vi "TCT .vi"(11 "VISA resource name":refnum<visa-resource-name>) -> ()   [LabVIEW 2016]
uses:
  <vilib>/NI/Modbus Library/API/Wrapper/Create Serial Master.vi
  <vilib>/NI/Modbus Library/API/Master/Modbus Master.lvclass
  <vilib>/NI/Modbus Library/API/Wrapper/API Main.lvlib
panel:
  out "Mean Temp.":dbl
  out "Voltage":dbl
  in  "y":bool
  out "Average hot plate temp.":dbl
  out "Average cold plate temp.":dbl
  out "Average Thermal conductivity":dbl
  out "LHP":dbl
  out "UHP":dbl
  out "LCP":dbl
  out "UCP":dbl
  out "x < y? 3":bool
  out "x < y? 2":bool
  in  "upper and lower cold plate":dbl
  out "upper conductivity":dbl
  out "Lower conductivity":dbl
  in  "Thickness":u16
  out "current":u16
  out "x < y?":bool
  in  "set hot plate temp":dbl
  out "current":u16[](array[numeric])
  out "lower cold plate":dbl
  out "lower hot plate":dbl
  out "upper hot plate":dbl
  out "upper cold plate":dbl
  out "element 13":u16
  out "element 12":u16
  out "element 11":u16
  out "element 10":u16
  out "element 9":u16
  out "element 8":u16
  out "element 7":u16
  out "element 6":u16
  out "element 5":u16
  out "element 4":u16
  out "element 3":u16
  out "element 2":u16
  out "voltage":u16
  out "register values 13":u16[](array[numeric])
  out "register values 12":u16[](array[numeric])
  out "register values 11":u16[](array[numeric])
  out "register values 10":u16[](array[numeric])
  out "register values 9":u16[](array[numeric])
  out "register values 8":u16[](array[numeric])
  out "register values 7":u16[](array[numeric])
  out "register values 6":u16[](array[numeric])
  out "register values 5":u16[](array[numeric])
  out "register values 4":u16[](array[numeric])
  out "register values 3":u16[](array[numeric])
  out "register values 2":u16[](array[numeric])
  out "register values":u16[](array[numeric])
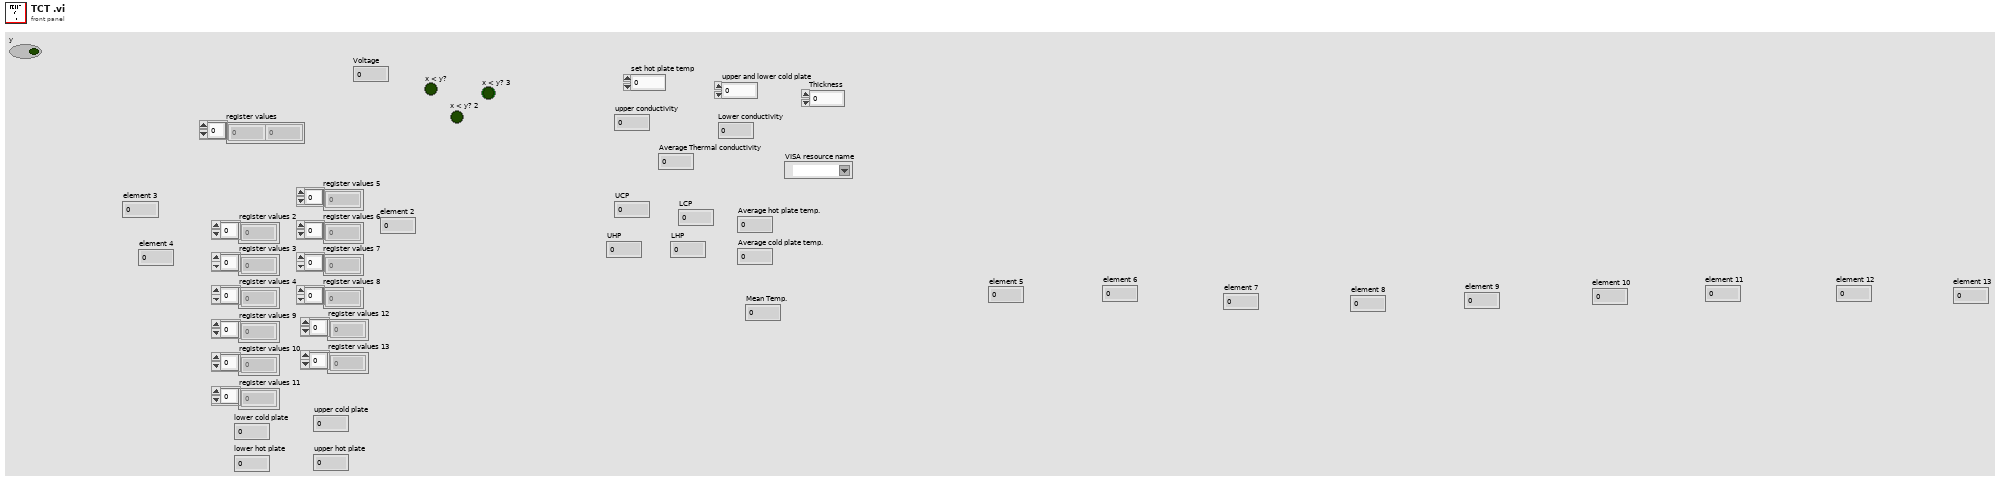
[diagram p1: front panel]
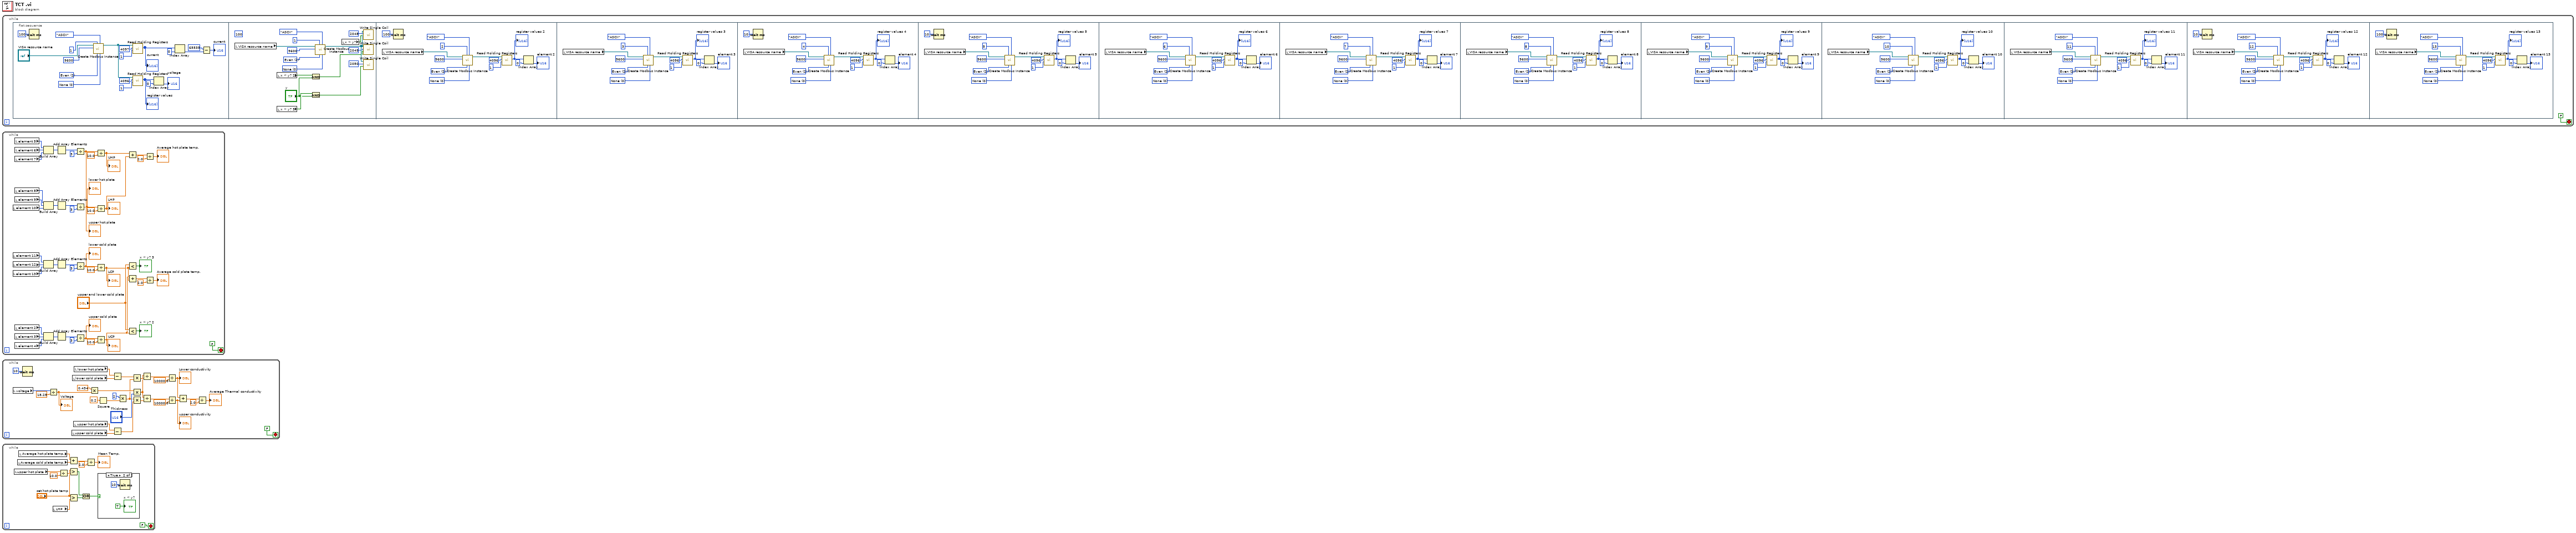
[diagram p0: block diagram]
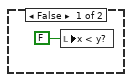
[diagram p2: hidden frame]
diagram:
  n1 = while {
    stop <- FALSE stop-if-true
    n2 = flat-sequence {
      frame #0 {
        w17 = u16 0 items=["None", "XON/XOFF", "RTS/CTS", "XON/XOFF & RTS/CTS", "DTR/DSR", "XON/XOFF & DTR/DSR"] ("flow control (none)")
        w18 = u16 2 items=["None", "Odd", "Even", "Mark", "Space"] ("parity (even)")
        n3 = Wait (ms)(milliseconds to wait=u32 100) -> ()  [unwired: 1 out]
        n4 = call-poly <vilib>:"Create Modbus Instance.vi"("flow control (none)"=w17, "serial type"=enum16{"RTU", "ASCII"}."ASCII", "parity (even)"=w18, "unit ID"=u8 1, "baud rate"=u32 9600, "VISA resource name"="VISA resource name") -> ("serial master instance"=w10:refnum<class "Modbus Master.lvclass">)  [unwired: 4 in, 1 out]
        n5 = call-dynamic "Read Holding Registers.vi"("number of inputs"=u16 1, "starting address"=u16 4097, "Modbus master in"=w10) -> ("register values"=w7:u16[])  [unwired: 6 in, 2 out]
        "current" <- w7
        n6 = call-dynamic "Read Holding Registers.vi"("number of inputs"=u16 1, "starting address"=u16 4096, "Modbus master in"=w10) -> ("register values"=w13:u16[])  [unwired: 6 in, 2 out]
        "register values" <- w13
        n7 = Index Array(array=w13, index=0) -> (element=→"voltage":u16)
        n8 = Index Array(array=w7, index=0) -> (element=w5:u16)
        n9 = Subtract(x=u16 65535, y=w5) -> (x-y=→"current":u16)
      }
      frame #1 {
        (unwired) u32 100 ("milliseconds to wait")
        w37 = u16 0 items=["None", "XON/XOFF", "RTS/CTS", "XON/XOFF & RTS/CTS", "DTR/DSR", "XON/XOFF & DTR/DSR"] ("flow control (none)")
        w36 = u16 2 items=["None", "Odd", "Even", "Mark", "Space"] ("parity (even)")
        n10 = local read "VISA resource name"() -> (w32:refnum<visa-resource-name>)
        n11 = local read "x < y? 2"() -> (w26:bool)
        n12 = local read "x < y? 3"() -> (w24:bool)
        n13 = And(x=w26, y="y") -> (x .and. y?=w25:bool)
        n14 = And(x=w24, y="y") -> (x .and. y?=w22:bool)
        n15 = call-poly <vilib>:"Create Modbus Instance.vi"("flow control (none)"=w37, "serial type"=enum16{"RTU", "ASCII"}."ASCII", "parity (even)"=w36, "unit ID"=u8 1, "baud rate"=u32 9600, "VISA resource name"=w32) -> ("serial master instance"=w30:refnum<class "Modbus Master.lvclass">)  [unwired: 4 in, 1 out]
        n16 = local read "x < y?"() -> (w27:bool)
        n17 = call-dynamic "Write Single Coil.vi"("coil to write"=w27, "address"=u16 2048, "Modbus master in"=w30) -> ()  [unwired: 7 in, 2 out]
        n18 = call-dynamic "Write Single Coil.vi"("coil to write"=w25, "address"=u16 2049, "Modbus master in"=w30) -> ()  [unwired: 7 in, 2 out]
        n19 = call-dynamic "Write Single Coil.vi"("coil to write"=w22, "address"=u16 2050, "Modbus master in"=w30) -> ()  [unwired: 7 in, 2 out]
      }
      frame #2 {
        w46 = u16 0 items=["None", "XON/XOFF", "RTS/CTS", "XON/XOFF & RTS/CTS", "DTR/DSR", "XON/XOFF & DTR/DSR"] ("flow control (none)")
        w47 = u16 2 items=["None", "Odd", "Even", "Mark", "Space"] ("parity (even)")
        n20 = local read "VISA resource name"() -> (w45:refnum<visa-resource-name>)
        n21 = Wait (ms)(milliseconds to wait=u32 100) -> ()  [unwired: 1 out]
        n22 = call-poly <vilib>:"Create Modbus Instance.vi"("flow control (none)"=w46, "serial type"=enum16{"RTU", "ASCII"}."ASCII", "parity (even)"=w47, "unit ID"=u8 2, "baud rate"=u32 9600, "VISA resource name"=w45) -> ("serial master instance"=w44:refnum<class "Modbus Master.lvclass">)  [unwired: 4 in, 1 out]
        n23 = call-dynamic "Read Holding Registers.vi"("number of inputs"=u16 1, "starting address"=u16 4096, "Modbus master in"=w44) -> ("register values"=w40:u16[])  [unwired: 6 in, 2 out]
        "register values 2" <- w40
        n24 = Index Array(array=w40, index=0) -> (element=→"element 2":u16)
      }
      frame #3 {
        w58 = u16 0 items=["None", "XON/XOFF", "RTS/CTS", "XON/XOFF & RTS/CTS", "DTR/DSR", "XON/XOFF & DTR/DSR"] ("flow control (none)")
        w59 = u16 2 items=["None", "Odd", "Even", "Mark", "Space"] ("parity (even)")
        n25 = local read "VISA resource name"() -> (w57:refnum<visa-resource-name>)
        n26 = call-poly <vilib>:"Create Modbus Instance.vi"("flow control (none)"=w58, "serial type"=enum16{"RTU", "ASCII"}."ASCII", "parity (even)"=w59, "unit ID"=u8 3, "baud rate"=u32 9600, "VISA resource name"=w57) -> ("serial master instance"=w56:refnum<class "Modbus Master.lvclass">)  [unwired: 4 in, 1 out]
        n27 = call-dynamic "Read Holding Registers.vi"("number of inputs"=u16 1, "starting address"=u16 4096, "Modbus master in"=w56) -> ("register values"=w52:u16[])  [unwired: 6 in, 2 out]
        "register values 3" <- w52
        n28 = Index Array(array=w52, index=0) -> (element=→"element 3":u16)
      }
      frame #4 {
        w75 = u16 0 items=["None", "XON/XOFF", "RTS/CTS", "XON/XOFF & RTS/CTS", "DTR/DSR", "XON/XOFF & DTR/DSR"] ("flow control (none)")
        w74 = u16 2 items=["None", "Odd", "Even", "Mark", "Space"] ("parity (even)")
        n29 = local read "VISA resource name"() -> (w70:refnum<visa-resource-name>)
        n30 = Wait (ms)(milliseconds to wait=u32 10) -> ()  [unwired: 1 out]
        n31 = call-poly <vilib>:"Create Modbus Instance.vi"("flow control (none)"=w75, "serial type"=enum16{"RTU", "ASCII"}."ASCII", "parity (even)"=w74, "unit ID"=u8 4, "baud rate"=u32 9600, "VISA resource name"=w70) -> ("serial master instance"=w65:refnum<class "Modbus Master.lvclass">)  [unwired: 4 in, 1 out]
        n32 = call-dynamic "Read Holding Registers.vi"("number of inputs"=u16 1, "starting address"=u16 4096, "Modbus master in"=w65) -> ("register values"=w67:u16[])  [unwired: 6 in, 2 out]
        "register values 4" <- w67
        n33 = Index Array(array=w67, index=0) -> (element=→"element 4":u16)
      }
      frame #5 {
        w88 = u16 0 items=["None", "XON/XOFF", "RTS/CTS", "XON/XOFF & RTS/CTS", "DTR/DSR", "XON/XOFF & DTR/DSR"] ("flow control (none)")
        w87 = u16 2 items=["None", "Odd", "Even", "Mark", "Space"] ("parity (even)")
        n34 = local read "VISA resource name"() -> (w83:refnum<visa-resource-name>)
        n35 = Wait (ms)(milliseconds to wait=u32 10) -> ()  [unwired: 1 out]
        n36 = call-poly <vilib>:"Create Modbus Instance.vi"("flow control (none)"=w88, "serial type"=enum16{"RTU", "ASCII"}."ASCII", "parity (even)"=w87, "unit ID"=u8 5, "baud rate"=u32 9600, "VISA resource name"=w83) -> ("serial master instance"=w81:refnum<class "Modbus Master.lvclass">)  [unwired: 4 in, 1 out]
        n37 = call-dynamic "Read Holding Registers.vi"("number of inputs"=u16 1, "starting address"=u16 4096, "Modbus master in"=w81) -> ("register values"=w78:u16[])  [unwired: 6 in, 2 out]
        "register values 5" <- w78
        n38 = Index Array(array=w78, index=0) -> (element=→"element 5":u16)
      }
      frame #6 {
        w100 = u16 0 items=["None", "XON/XOFF", "RTS/CTS", "XON/XOFF & RTS/CTS", "DTR/DSR", "XON/XOFF & DTR/DSR"] ("flow control (none)")
        w99 = u16 2 items=["None", "Odd", "Even", "Mark", "Space"] ("parity (even)")
        n39 = local read "VISA resource name"() -> (w95:refnum<visa-resource-name>)
        n40 = call-poly <vilib>:"Create Modbus Instance.vi"("flow control (none)"=w100, "serial type"=enum16{"RTU", "ASCII"}."ASCII", "parity (even)"=w99, "unit ID"=u8 6, "baud rate"=u32 9600, "VISA resource name"=w95) -> ("serial master instance"=w93:refnum<class "Modbus Master.lvclass">)  [unwired: 4 in, 1 out]
        n41 = call-dynamic "Read Holding Registers.vi"("number of inputs"=u16 1, "starting address"=u16 4096, "Modbus master in"=w93) -> ("register values"=w90:u16[])  [unwired: 6 in, 2 out]
        "register values 6" <- w90
        n42 = Index Array(array=w90, index=0) -> (element=→"element 6":u16)
      }
      frame #7 {
        w108 = u16 0 items=["None", "XON/XOFF", "RTS/CTS", "XON/XOFF & RTS/CTS", "DTR/DSR", "XON/XOFF & DTR/DSR"] ("flow control (none)")
        w109 = u16 2 items=["None", "Odd", "Even", "Mark", "Space"] ("parity (even)")
        n43 = local read "VISA resource name"() -> (w107:refnum<visa-resource-name>)
        n44 = call-poly <vilib>:"Create Modbus Instance.vi"("flow control (none)"=w108, "serial type"=enum16{"RTU", "ASCII"}."ASCII", "parity (even)"=w109, "unit ID"=u8 7, "baud rate"=u32 9600, "VISA resource name"=w107) -> ("serial master instance"=w106:refnum<class "Modbus Master.lvclass">)  [unwired: 4 in, 1 out]
        n45 = call-dynamic "Read Holding Registers.vi"("number of inputs"=u16 1, "starting address"=u16 4096, "Modbus master in"=w106) -> ("register values"=w101:u16[])  [unwired: 6 in, 2 out]
        "register values 7" <- w101
        n46 = Index Array(array=w101, index=0) -> (element=→"element 7":u16)
      }
      frame #8 {
        w124 = u16 0 items=["None", "XON/XOFF", "RTS/CTS", "XON/XOFF & RTS/CTS", "DTR/DSR", "XON/XOFF & DTR/DSR"] ("flow control (none)")
        w123 = u16 2 items=["None", "Odd", "Even", "Mark", "Space"] ("parity (even)")
        n47 = local read "VISA resource name"() -> (w119:refnum<visa-resource-name>)
        n48 = call-poly <vilib>:"Create Modbus Instance.vi"("flow control (none)"=w124, "serial type"=enum16{"RTU", "ASCII"}."ASCII", "parity (even)"=w123, "unit ID"=u8 8, "baud rate"=u32 9600, "VISA resource name"=w119) -> ("serial master instance"=w118:refnum<class "Modbus Master.lvclass">)  [unwired: 4 in, 1 out]
        n49 = call-dynamic "Read Holding Registers.vi"("number of inputs"=u16 1, "starting address"=u16 4096, "Modbus master in"=w118) -> ("register values"=w114:u16[])  [unwired: 6 in, 2 out]
        "register values 8" <- w114
        n50 = Index Array(array=w114, index=0) -> (element=→"element 8":u16)
      }
      frame #9 {
        w132 = u16 0 items=["None", "XON/XOFF", "RTS/CTS", "XON/XOFF & RTS/CTS", "DTR/DSR", "XON/XOFF & DTR/DSR"] ("flow control (none)")
        w133 = u16 2 items=["None", "Odd", "Even", "Mark", "Space"] ("parity (even)")
        n51 = local read "VISA resource name"() -> (w131:refnum<visa-resource-name>)
        n52 = call-poly <vilib>:"Create Modbus Instance.vi"("flow control (none)"=w132, "serial type"=enum16{"RTU", "ASCII"}."ASCII", "parity (even)"=w133, "unit ID"=u8 9, "baud rate"=u32 9600, "VISA resource name"=w131) -> ("serial master instance"=w130:refnum<class "Modbus Master.lvclass">)  [unwired: 4 in, 1 out]
        n53 = call-dynamic "Read Holding Registers.vi"("number of inputs"=u16 1, "starting address"=u16 4096, "Modbus master in"=w130) -> ("register values"=w125:u16[])  [unwired: 6 in, 2 out]
        "register values 9" <- w125
        n54 = Index Array(array=w125, index=0) -> (element=→"element 9":u16)
      }
      frame #10 {
        w144 = u16 0 items=["None", "XON/XOFF", "RTS/CTS", "XON/XOFF & RTS/CTS", "DTR/DSR", "XON/XOFF & DTR/DSR"] ("flow control (none)")
        w145 = u16 2 items=["None", "Odd", "Even", "Mark", "Space"] ("parity (even)")
        n55 = local read "VISA resource name"() -> (w143:refnum<visa-resource-name>)
        n56 = call-poly <vilib>:"Create Modbus Instance.vi"("flow control (none)"=w144, "serial type"=enum16{"RTU", "ASCII"}."ASCII", "parity (even)"=w145, "unit ID"=u8 10, "baud rate"=u32 9600, "VISA resource name"=w143) -> ("serial master instance"=w142:refnum<class "Modbus Master.lvclass">)  [unwired: 4 in, 1 out]
        n57 = call-dynamic "Read Holding Registers.vi"("number of inputs"=u16 1, "starting address"=u16 4096, "Modbus master in"=w142) -> ("register values"=w137:u16[])  [unwired: 6 in, 2 out]
        "register values 10" <- w137
        n58 = Index Array(array=w137, index=0) -> (element=→"element 10":u16)
      }
      frame #11 {
        w160 = u16 0 items=["None", "XON/XOFF", "RTS/CTS", "XON/XOFF & RTS/CTS", "DTR/DSR", "XON/XOFF & DTR/DSR"] ("flow control (none)")
        w159 = u16 2 items=["None", "Odd", "Even", "Mark", "Space"] ("parity (even)")
        n59 = local read "VISA resource name"() -> (w155:refnum<visa-resource-name>)
        n60 = call-poly <vilib>:"Create Modbus Instance.vi"("flow control (none)"=w160, "serial type"=enum16{"RTU", "ASCII"}."ASCII", "parity (even)"=w159, "unit ID"=u8 11, "baud rate"=u32 9600, "VISA resource name"=w155) -> ("serial master instance"=w154:refnum<class "Modbus Master.lvclass">)  [unwired: 4 in, 1 out]
        n61 = call-dynamic "Read Holding Registers.vi"("number of inputs"=u16 1, "starting address"=u16 4096, "Modbus master in"=w154) -> ("register values"=w149:u16[])  [unwired: 6 in, 2 out]
        "register values 11" <- w149
        n62 = Index Array(array=w149, index=0) -> (element=→"element 11":u16)
      }
      frame #12 {
        w169 = u16 0 items=["None", "XON/XOFF", "RTS/CTS", "XON/XOFF & RTS/CTS", "DTR/DSR", "XON/XOFF & DTR/DSR"] ("flow control (none)")
        w170 = u16 2 items=["None", "Odd", "Even", "Mark", "Space"] ("parity (even)")
        n63 = local read "VISA resource name"() -> (w168:refnum<visa-resource-name>)
        n64 = Wait (ms)(milliseconds to wait=u32 10) -> ()  [unwired: 1 out]
        n65 = call-poly <vilib>:"Create Modbus Instance.vi"("flow control (none)"=w169, "serial type"=enum16{"RTU", "ASCII"}."ASCII", "parity (even)"=w170, "unit ID"=u8 12, "baud rate"=u32 9600, "VISA resource name"=w168) -> ("serial master instance"=w167:refnum<class "Modbus Master.lvclass">)  [unwired: 4 in, 1 out]
        n66 = call-dynamic "Read Holding Registers.vi"("number of inputs"=u16 1, "starting address"=u16 4096, "Modbus master in"=w167) -> ("register values"=w162:u16[])  [unwired: 6 in, 2 out]
        "register values 12" <- w162
        n67 = Index Array(array=w162, index=0) -> (element=→"element 12":u16)
      }
      frame #13 {
        w182 = u16 0 items=["None", "XON/XOFF", "RTS/CTS", "XON/XOFF & RTS/CTS", "DTR/DSR", "XON/XOFF & DTR/DSR"] ("flow control (none)")
        w183 = u16 2 items=["None", "Odd", "Even", "Mark", "Space"] ("parity (even)")
        n68 = local read "VISA resource name"() -> (w181:refnum<visa-resource-name>)
        n69 = Wait (ms)(milliseconds to wait=u32 100) -> ()  [unwired: 1 out]
        n70 = call-poly <vilib>:"Create Modbus Instance.vi"("flow control (none)"=w182, "serial type"=enum16{"RTU", "ASCII"}."ASCII", "parity (even)"=w183, "unit ID"=u8 13, "baud rate"=u32 9600, "VISA resource name"=w181) -> ("serial master instance"=w180:refnum<class "Modbus Master.lvclass">)  [unwired: 4 in, 1 out]
        n71 = call-dynamic "Read Holding Registers.vi"("number of inputs"=u16 1, "starting address"=u16 4096, "Modbus master in"=w180) -> ("register values"=w175:u16[])  [unwired: 6 in, 2 out]
        "register values 13" <- w175
        n72 = Index Array(array=w175, index=0) -> (element=→"element 13":u16)
      }
    }
  }
  n73 = while {
    stop <- FALSE stop-if-true
    n74 = local read "element 10"() -> (w217:u16)
    n75 = local read "element 11"() -> (w213:u16)
    n76 = local read "element 12"() -> (w212:u16)
    n77 = local read "element 13"() -> (w211:u16)
    n78 = local read "element 5"() -> (w225:u16)
    n79 = local read "element 6"() -> (w224:u16)
    n80 = local read "element 7"() -> (w223:u16)
    n81 = local read "element 8"() -> (w219:u16)
    n82 = local read "element 9"() -> (w218:u16)
    n83 = local read "element 2"() -> (w231:u16)
    n84 = local read "element 3"() -> (w230:u16)
    n85 = local read "element 4"() -> (w229:u16)
    n86 = Build Array(w225, w224, w223) -> (w222:u16[])
    n87 = Build Array(w219, w218, w217) -> (w216:u16[])
    n88 = Build Array(w213, w212, w211) -> (w210:u16[])
    n89 = Build Array(w231, w230, w229) -> (w228:u16[])
    n90 = Add Array Elements(numeric array=w222) -> (sum=w221:u16)
    n91 = Add Array Elements(numeric array=w216) -> (sum=w215:u16)
    n92 = Add Array Elements(numeric array=w210) -> (sum=w209:u16)
    n93 = Add Array Elements(numeric array=w228) -> (sum=w227:u16)
    n94 = Divide(x=w221, y=u16 3) -> (x/y=w192:dbl)
    "upper hot plate" <- w192
    n95 = Divide(x=w215, y=u16 3) -> (x/y=w199:dbl)
    "lower hot plate" <- w199
    n96 = Divide(x=w209, y=u16 3) -> (x/y=w205:dbl)
    "lower cold plate" <- w205
    n97 = Divide(x=w227, y=u16 3) -> (x/y=w206:dbl)
    "upper cold plate" <- w206
    n98 = Divide(x=w192, y=10.0) -> (x/y=w191:dbl)
    "UHP" <- w191
    n99 = Divide(x=w199, y=10.0) -> (x/y=w190:dbl)
    "LHP" <- w190
    n100 = Divide(x=w205, y=10.0) -> (x/y=w196:dbl)
    "LCP" <- w196
    n101 = Divide(x=w206, y=10.0) -> (x/y=w197:dbl)
    "UCP" <- w197
    n102 = Add(x=w191, y=w190) -> (x+y=w189:dbl)
    n103 = Less?(x="upper and lower cold plate", y=w196) -> (x < y?=→"x < y? 3":bool)
    n104 = Add(x=w197, y=w196) -> (x+y=w195:dbl)
    n105 = Less?(x="upper and lower cold plate", y=w197) -> (x < y?=→"x < y? 2":bool)
    n106 = Divide(x=w189, y=2.0) -> (x/y=→"Average hot plate temp.":dbl)
    n107 = Divide(x=w195, y=2.0) -> (x/y=→"Average cold plate temp.":dbl)
  }
  n108 = while {
    stop <- FALSE stop-if-true
    n109 = local read "voltage"() -> (w242:u16)
    n110 = Wait (ms)(milliseconds to wait=u32 10) -> ()  [unwired: 1 out]
    n111 = Divide(x=w242, y=18.25) -> (x/y=w240:dbl)
    "Voltage" <- w240
    n112 = local read "upper cold plate"() -> (w253:dbl)
    n113 = local read "lower cold plate"() -> (w255:dbl)
    n114 = local read "upper hot plate"() -> (w254:dbl)
    n115 = local read "lower hot plate"() -> (w256:dbl)
    n116 = Multiply(x=0.434, y=w240) -> (x*y=w261:dbl)
    n117 = Square(x=0.2) -> (x^2=w257:dbl)
    n118 = Subtract(x=w256, y=w255) -> (x-y=w252:dbl)
    n119 = Subtract(x=w254, y=w253) -> (x-y=w250:dbl)
    n120 = Multiply(x=2, y=w257) -> (x*y=w251:dbl)
    n121 = Multiply(x=w252, y=w251) -> (x*y=w249:dbl)
    n122 = Multiply(x=w261, y="Thickness") -> (x*y=w248:dbl)
    n123 = Multiply(x=w251, y=w250) -> (x*y=w247:dbl)
    n124 = Divide(x=w248, y=w249) -> (x/y=w246:dbl)
    n125 = Divide(x=w248, y=w247) -> (x/y=w244:dbl)
    n126 = Divide(x=w246, y=10000.0) -> (x/y=w238:dbl)
    "Lower conductivity" <- w238
    n127 = Divide(x=w244, y=10000.0) -> (x/y=w237:dbl)
    "upper conductivity" <- w237
    n128 = Add(x=w238, y=w237) -> (x+y=w236:dbl)
    n129 = Divide(x=w236, y=2.0) -> (x/y=→"Average Thermal conductivity":dbl)
  }
  n130 = while {
    stop <- FALSE stop-if-true
    n131 = local read "upper hot plate"() -> (w274:dbl)
    n132 = local read "Average cold plate temp."() -> (w266:dbl)
    n133 = local read "Average hot plate temp."() -> (w267:dbl)
    n134 = local read "LHP"() -> (w271:dbl)
    n135 = Divide(x=w274, y=10.0) -> (x/y=w275:dbl)
    n136 = Add(x=w267, y=w266) -> (x+y=w265:dbl)
    n137 = Greater?(x="set hot plate temp", y=w275) -> (0:w272:bool)
    n138 = Greater?(x="set hot plate temp", y=w271) -> (0:w269:bool)
    n139 = Or(x=w272, y=w269) -> (x .or. y?=w268:bool)
    n140 = Divide(x=w265, y=2.0) -> (x/y=→"Mean Temp.":dbl)
    n141 = case shown="True" w268 {
      frame False {
        n142 = local write "x < y?"(FALSE ("x < y?")) -> ()
      }
      frame True {
        n143 = Wait (ms)(milliseconds to wait=u32 10) -> ()  [unwired: 1 out]
        "x < y?" <- TRUE ("x < y?")
      }
    }
  }
